vi "Add Item to Virtual Folder.vi"(8 "error in":errorcluster, 9 "File Path":path, 10 "Virtual Folder":string, 11 "Project Manager in":refnum<class "Project Manager.lvclass">) -> (0 "error out":errorcluster, 3 "Project Manager out":refnum<class "Project Manager.lvclass">)   [LabVIEW 2026, in "Project Manager.lvclass"]
doc: "Add file to a virtual folder specified by name."
uses:
  Project Manager.lvclass
  Project Manager.lvclass/Project Manager.ctl
  <vilib>/ActorFramework/Message Enqueuer/Message Enqueuer.lvclass
  Interfaces/ILogger/ILogger Messages/Log Msg/Log Msg.lvclass
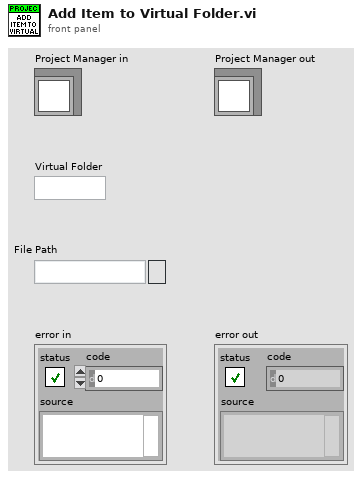
[diagram p1: front panel]
types:
  T1 = typedef "Log Entry--cluster.ctl" = cluster{"Time":timestamp, "Message":string}
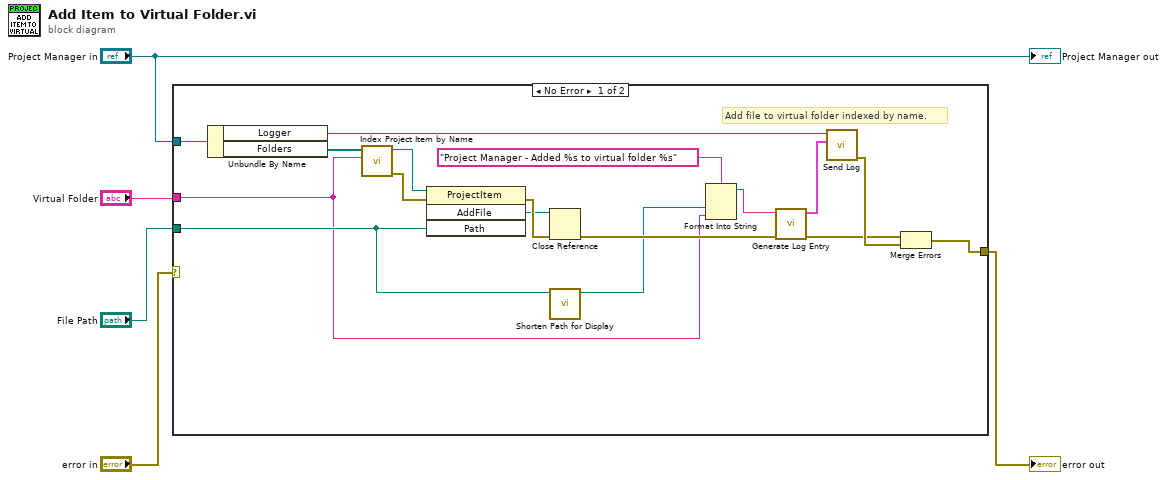
[diagram p0: block diagram]
diagram:
  n1 = case shown="No Error" "error in" {
    selector: "error in" -> [_ w23]
    tunnel: "Project Manager in" -> [w16 _]
    tunnel: "File Path" -> [w9 _]
    tunnel: [w20 w23] -> w4
    tunnel: "Virtual Folder" -> [w7 _]
    frame No Error {
      # "Add file to virtual folder indexed by name."
      n2 = Unbundle By Name(w16) -> ("Logger"=w12:refnum<class "Message Enqueuer.lvclass">, "Folders"=w14:refnum<vi>[])
      n3 = call "Index Project Item by Name.vi"("Name"=w7, "Project Items"=w14) -> ("error out"=w21:errorcluster, "Project Item"=w13:refnum<vi>)  [unwired: 8 in]
      n4 = invoke class="ProjectItem" method="AddFile"(reference=w13, error in=w21, "Path"=w9) -> (error out=w22:errorcluster, "AddFile"=w15:refnum<vi>)  [unwired: 1 in, 2 out]
      n5 = Close Reference(reference=w15, error in (no error)=w22) -> (error out=w18:errorcluster)
      n6 = call "Shorten Path for Display.vi"("Path"=w9) -> ("Shortened Path"=w8:path)  [unwired: 10 in]
      n7 = Format Into String(format string="Project Manager - Added %s to virtual folder %s", w8, w7) -> (resulting string=w6:string)  [unwired: 2 in, 1 out]
      n8 = call "Generate Log Entry.vi"("error in"=w18, "Message"=w6) -> ("error out"=w17:errorcluster, "Log Entry"=w11:T1)  [unwired: 8 in]
      n9 = call "Send Log.vi"("Log Entry"=w11, "Message Enqueuer"=w12) -> ("error out"=w19:errorcluster)  [unwired: 8 in, 1 out]
      n10 = Merge Errors(w17, w19) -> (w20:errorcluster)
    }
    frame Error {
      # "Pass error without further action."
    }
  }
  "error out" <- w4
  "Project Manager out" <- "Project Manager in"
